vi "Open CSM_Tool_Launcher.vi"() -> ()   [LabVIEW 2017, in "csm_tool_menu.lvlib"]
uses:
  csm_tool_menu.lvlib
  fd0165b5-6fc4-4d2a-af44-7735b0eff26e.vi
  user.lib/_NEVSTOP/Communicable State Machine(CSM)/_xnode/csm_tool/_xnode_csm_tool_support/CSM DebugTool Dialog.lvlib
  user.lib/_NEVSTOP/Communicable State Machine(CSM)/_tool/_ui/csm-ui-support.lvlib
panel:
  in  "error in (no error)":errorcluster
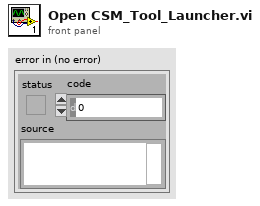
[diagram p1: front panel]
types:
  T1 = enum32{"Invalid", "Standard", "Closed", "Hidden", "Minimized", "Maximized"}
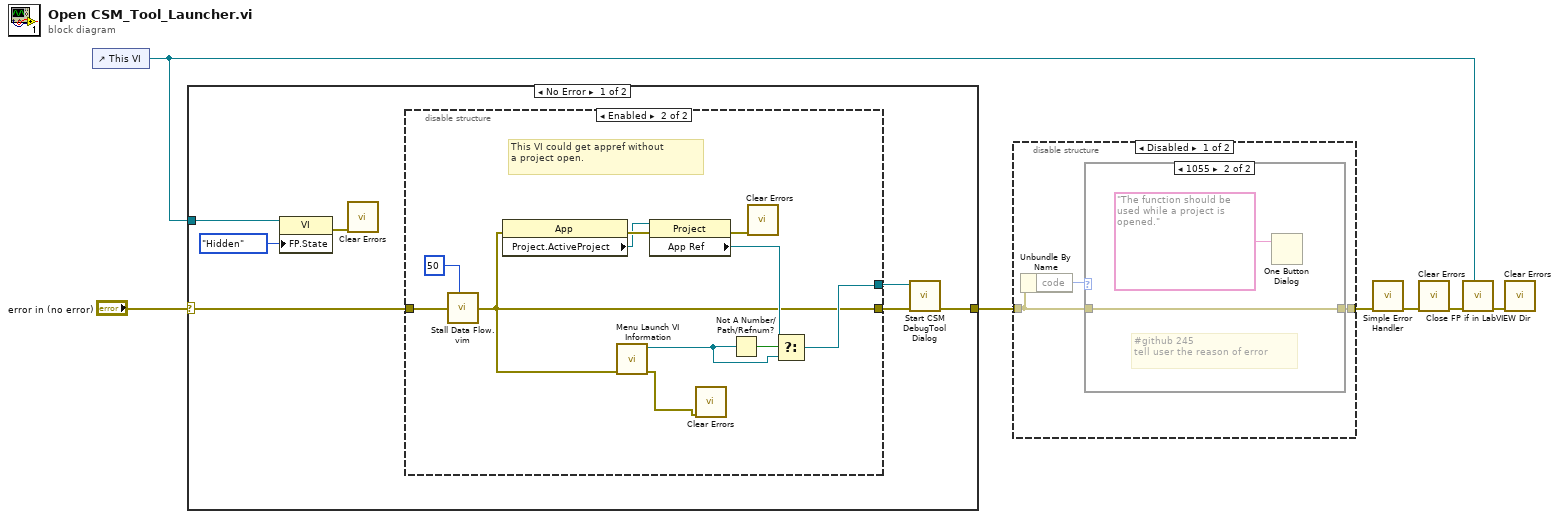
[diagram p0: block diagram]
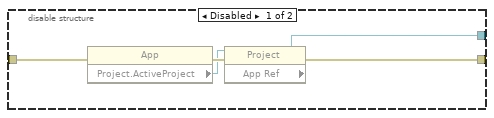
[diagram p2: hidden frame]
diagram:
  n1 = control-ref of="This VI"() -> (w1:refnum<vi>)
  n2 = case shown="No Error" "error in (no error)" {
    selector: "error in (no error)" -> [w14 w31]
    tunnel: [w11 w31] -> w3
    tunnel: w1 -> [w10 _]
    frame No Error {
      n3 = property class="VI"(reference=w10, "FP.State"=T1."Hidden" ("Front Panel Window:State")) -> (error out=w8:errorcluster)  [unwired: 1 in, 1 out]
      n4 = call <vilib>:"Clear Errors.vi"("error in (no error)"=w8) -> ()  [unwired: 5 in, 2 out]
      n5 = disable-structure shown="Enabled" {
        disable-tunnel: w14 -> [w19 w24]
        disable-tunnel: [w16 w21] -> w13
        disable-tunnel: [w15 w25] -> w12
        frame Disabled {
          n6 = property class="App"(error in=w19) -> (error out=w18:errorcluster, "Project.ActiveProject"=w17:refnum<vi>)  [unwired: 1 in, 1 out]
          n7 = property class="Project"(reference=w17, error in=w18) -> (error out=w16:errorcluster, "App Ref"=w15:refnum<vi>)  [unwired: 1 out]
        }
        frame Enabled {
          # "This VI could get appref without \na project open."
          n8 = call "Stall Data Flow.vim"("value in"=w24, "milliseconds to wait"=u32 50) -> ("value out"=w21:errorcluster)  [unwired: 1 out]
          n9 = property class="App"(error in=w21) -> (error out=w29:errorcluster, "Project.ActiveProject"=w28:refnum<vi>)  [unwired: 1 in, 1 out]
          n10 = call <vilib>:"Menu Launch VI Information.vi"("error in (no error)"=w21) -> ("error out"=w22:errorcluster, "Menu Launch:App"=w27:refnum<vi>)  [unwired: 8 in, 1 out]
          n11 = property class="Project"(reference=w28, error in=w29) -> (error out=w23:errorcluster, "App Ref"=w26:refnum<vi>)  [unwired: 1 out]
          n12 = call <vilib>:"Clear Errors.vi"("error in (no error)"=w22) -> ()  [unwired: 5 in, 2 out]
          n13 = Not A Number/Path/Refnum?(number/path/refnum=w27) -> (NaN/Path/Refnum?=w30:bool)
          n14 = call <vilib>:"Clear Errors.vi"("error in (no error)"=w23) -> ()  [unwired: 5 in, 2 out]
          n15 = Select(t=w26, s=w30, f=w27) -> (s? t:f=w25:refnum<vi>)
        }
      }
      n16 = call "Start CSM DebugTool Dialog.vi"("error in (no error)"=w13, "Application In"=w12) -> ("error out"=w11:errorcluster)  [unwired: 9 in]
    }
    frame Error {
    }
  }
  n17 = disable-structure shown="Disabled" {
    disable-tunnel: [w34 w38] -> w4
    disable-tunnel: w3 -> [w33 w38]
    frame Disabled {
      n18 = Unbundle By Name(w33) -> ("code"=w32:i32)
      n19 = case shown="1055" w32 {
        tunnel: w33 -> [w35 w37]
        tunnel: [w35 w37] -> w34
        frame 0, Default {
        }
        frame 1055 {
          # "#github 245\ntell user the reason of error"
          n20 = One Button Dialog(message="The function should be used while a project is opened.") -> ()  [unwired: 1 in, 1 out]
        }
      }
    }
    frame Enabled {
    }
  }
  n21 = call <vilib>:"Simple Error Handler.vi"("error in (no error)"=w4) -> ("error out"=w2:errorcluster)  [unwired: 4 in, 4 out]
  n22 = call <vilib>:"Clear Errors.vi"("error in (no error)"=w2) -> ("error out"=w6:errorcluster)  [unwired: 5 in, 1 out]
  n23 = call "Close FP if in LabVIEW Dir.vi"("VI Refnum"=w1, "Error in"=w6) -> ("Error out"=w7:errorcluster)  [unwired: 9 in]
  n24 = call <vilib>:"Clear Errors.vi"("error in (no error)"=w7) -> ()  [unwired: 5 in, 2 out]
